vi "Handshake.vi"(8 "error in (no error)":errorcluster, 11 "Connection.LocalQueue":refnum<class "Connection.LocalQueue.lvclass">) -> (0 "error out":errorcluster, 3 "Connection.LocalQueue":refnum<class "Connection.LocalQueue.lvclass">)   [LabVIEW 2013, in "Connection.Queue_GOSPL.lvlib" / "Connection.LocalQueue.lvclass"]
uses:
  Connection.LocalQueue.lvclass
  Connection/Connection.lvclass/Connection.ctl
  Connection/Connection.lvclass
  Connection.LocalQueue.lvclass/Connection.LocalQueue.ctl
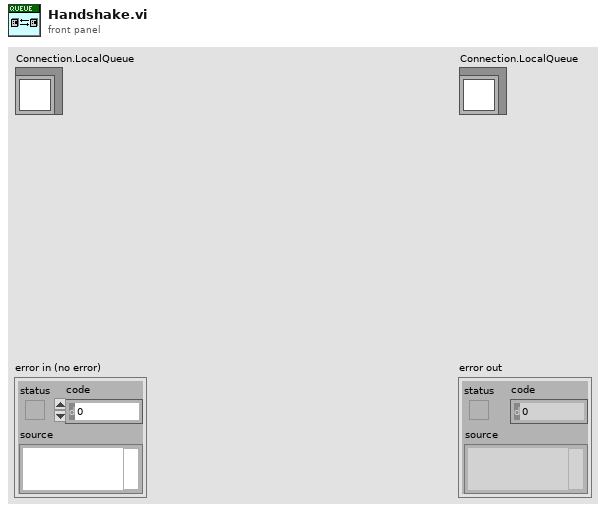
[diagram p1: front panel]
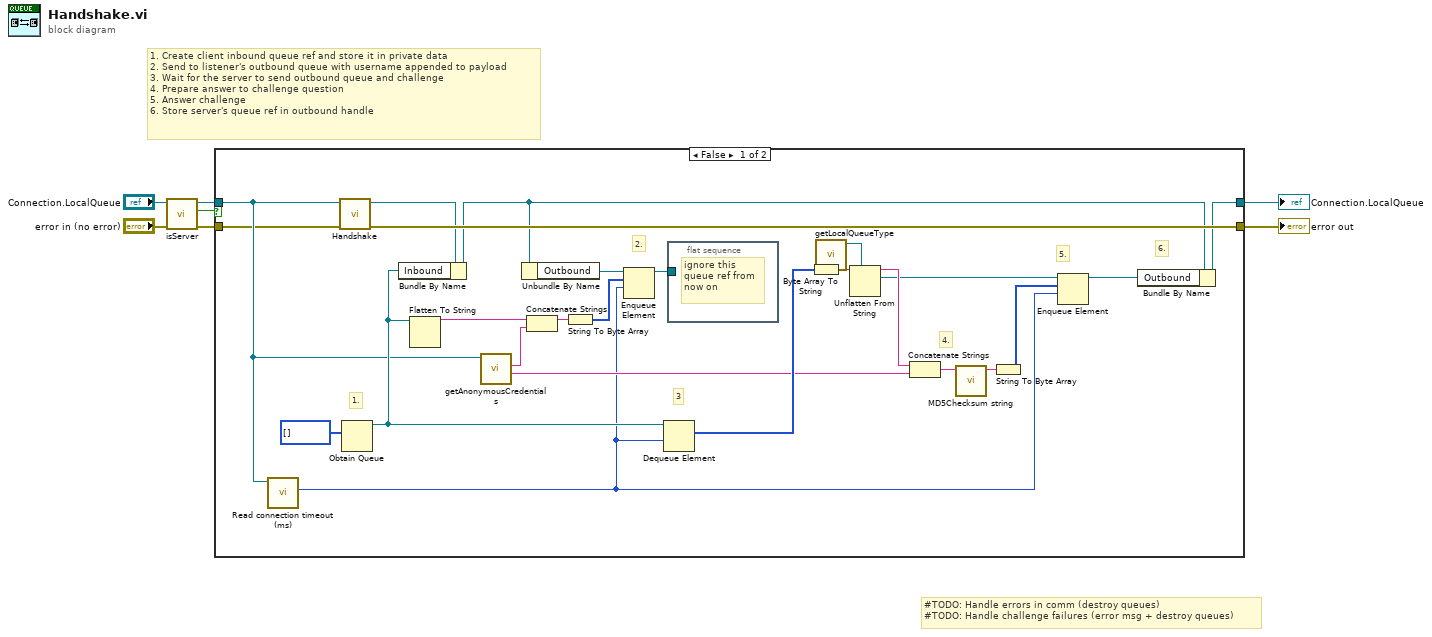
[diagram p0: block diagram]
diagram:
  # "#TODO: Handle errors in comm (destroy queues)\n#TODO: Handle challenge failures (error msg + destroy queues)"
  # "1. Create client inbound queue ref and store it in private data\n2. Send to listener's outbound queue with username appended to payload\n3. Wait for the server to send outbound queue and challenge\n4. Prepare answer to challenge question\n5. Answer challenge\n6. Store server's queue ref in outbound handle"
  n1 = call "isServer.vi"("error in (no error)"="error in (no error)", "Connection in"="Connection.LocalQueue") -> ("error out"=w2:errorcluster, "server"=w1:bool, "Connection out"=w4:refnum<class "Connection.LocalQueue.lvclass">)  [unwired: 7 in]
  n2 = case shown="False" w1 {
    tunnel: [w32 w33] -> w7
    tunnel: [w20 w34] -> w6
    tunnel: w4 -> [w9 w34]
    tunnel: w2 -> [w8 w33]
    frame False {
      # "6."
      # "5."
      # "4."
      # "3"
      # "2."
      # "1."
      n3 = call "Read connection timeout (ms).vi"("Connection in"=w9) -> ("connection timeout (ms)"=w10:i32)  [unwired: 8 in, 2 out]
      n4 = call-parent "Handshake.vi"("error in (no error)"=w8, "Connection in"=w9) -> ("error out"=w32:errorcluster, "Connection out"=w23:refnum<class "Connection.LocalQueue.lvclass">)  [unwired: 8 in]
      n5 = Obtain Queue(element data type=u8[] [] ("Bytes")) -> (queue out=w22:refnum<queue>)  [unwired: 4 in, 2 out]
      n6 = Bundle By Name(cluster=w23, "Inbound"=w22) -> (w21:refnum<class "Connection.LocalQueue.lvclass">)
      n7 = Flatten To String(anything=w22) -> (data string=w27:string)  [unwired: 3 in, 2 out]
      n8 = call "getAnonymousCredentials.vi"("Connection.LocalQueue"=w9) -> ("Anonymous password"=w16:string, "Anonymous username"=w28:string)  [unwired: 9 in]
      n9 = Unbundle By Name(w21) -> ("Outbound"=w30:refnum<queue>)
      n10 = Concatenate Strings(w27, w28) -> (w26:string)
      n11 = String To Byte Array(string=w26) -> (unsigned byte array=w29:u8[])
      n12 = Enqueue Element(queue=w30, element=w29, timeout in ms (-1)=w10) -> (queue out=w24:refnum<queue>)  [unwired: 1 in, 2 out]
      n13 = Dequeue Element(queue=w22, timeout in ms (-1)=w10) -> (element=w17:u8[])  [unwired: 1 in, 3 out]
      n14 = flat-sequence {
        tunnel: w24 -> [_]
        frame #0 {
          # "ignore this\nqueue ref from\nnow on"
        }
      }
      n15 = Byte Array To String(unsigned byte array=w17) -> (string=w18:string)
      n16 = call "getLocalQueueType.vi"() -> ("Queue Type"=w19:refnum<queue>)  [unwired: 11 in]
      n17 = Unflatten From String(type=w19, binary string=w18) -> (rest of the binary string=w15:string, value=w14:refnum<queue>)  [unwired: 3 in, 1 out]
      n18 = Concatenate Strings(w15, w16) -> (w25:string)
      n19 = call <vilib>:"MD5Checksum string.vi"("Message String"=w25) -> ("MD5 message-digest"=w12:string)  [unwired: 10 in]
      n20 = String To Byte Array(string=w12) -> (unsigned byte array=w11:u8[])
      n21 = Enqueue Element(queue=w14, element=w11, timeout in ms (-1)=w10) -> (queue out=w13:refnum<queue>)  [unwired: 1 in, 2 out]
      n22 = Bundle By Name(cluster=w21, "Outbound"=w13) -> (w20:refnum<class "Connection.LocalQueue.lvclass">)
    }
    frame True {
    }
  }
  "error out" <- w7
  "Connection.LocalQueue" <- w6
